vi "CIVI Initialize.vi"(11 "VISA Resource Name":refnum<visa-resource-name>) -> (0 "error out":errorcluster, 3 "VISA Session out":refnum<visa-resource-name>)   [LabVIEW 2026]
doc: "Opens a VISA connection to the CIVI SCPI gateway.\nEnables LF read termination (ASCII 10) and sets the I/O timeout to 10000 ms.\nReturns the open VISA session and error status.\nDoes not reset or identify the instrument.\nClose the session with CIVI Close.vi."
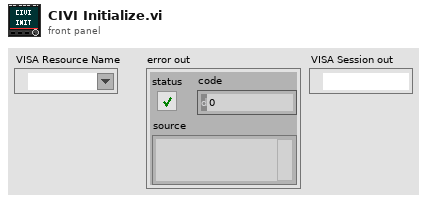
[diagram p1: front panel]
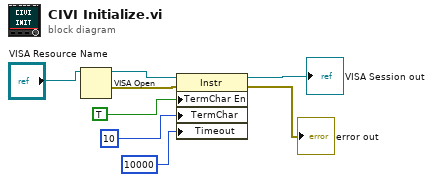
[diagram p0: block diagram]
diagram:
  n1 = VISA Open(VISA resource name="VISA Resource Name") -> (VISA resource name=w6:refnum<visa-resource-name>, error out=w5:errorcluster)  [unwired: 4 in]
  n2 = property class="Instr"(reference=w6, error in=w5, "TermChar En"=TRUE ("Message Based Settings:Termination Character Enable"), "TermChar"=u8 10 ("Message Based Settings:Termination Character"), "Timeout"=u32 10000 ("General Settings:Timeout Value")) -> (reference out=→"VISA Session out":refnum<visa-resource-name>, error out=→"error out":errorcluster)
